vi "Write Boolean.vi"(7 "RegisterOffset":u32, 8 "error in":errorcluster, 9 "value in":bool, 10 "register name":string, 11 "session in":u32) -> (0 "error out":errorcluster, 3 "session out":u32)   [LabVIEW 2020, in "FPGA Register IO.lvlib"]
uses:
  FPGA Register IO.lvlib
  NiFpga.dll
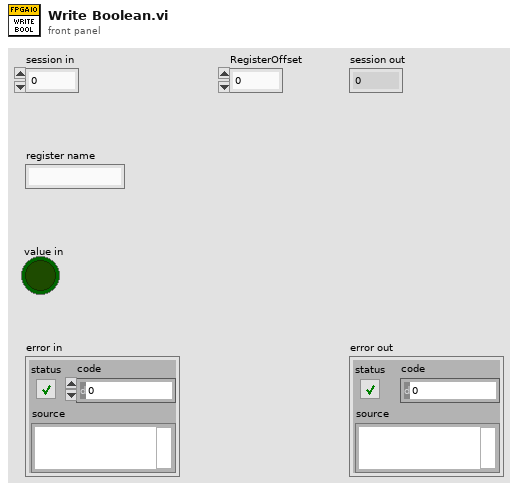
[diagram p1: front panel]
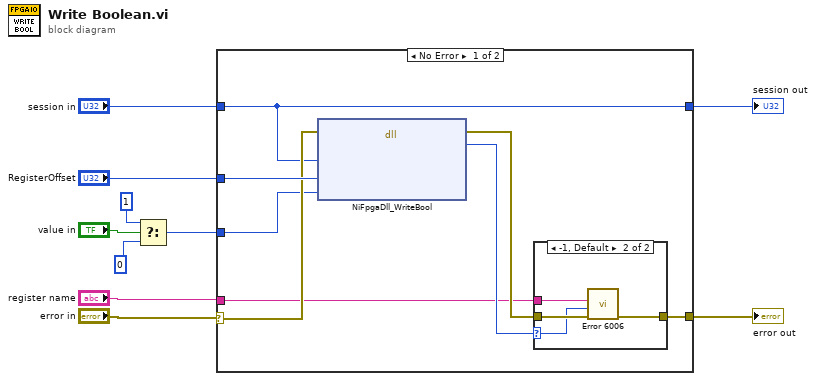
[diagram p0: block diagram]
diagram:
  n1 = Select(t=u8 1 ("value"), s="value in", f=u8 0) -> (s? t:f=w1:u8)
  n2 = case shown="No Error" "error in" {
    selector: "error in" -> [w17 w25]
    tunnel: "session in" -> [w16 w24]
    tunnel: [w11 w25] -> w10
    tunnel: "RegisterOffset" -> [w18 _]
    tunnel: [w16 w24] -> w9
    tunnel: w1 -> [w15 _]
    tunnel: "register name" -> [w12 _]
    frame No Error {
      n3 = dll-call lib="NiFpga.*" fn="NiFpgaDll_WriteBool"(error in=w17, "session"=w16, "offset"=w18, "value"=w15) -> (error out=w13:errorcluster, "status"=w14:i32)  [unwired: 5 in, 1 out]
      n4 = case shown="-1, Default" w14 {
        selector: w14 -> [_ w20]
        tunnel: w13 -> [w19 w21]
        tunnel: [w19 w23] -> w11
        tunnel: w12 -> [_ w22]
        frame 0 {
        }
        frame -1, Default {
          n5 = call "Error 6006.vi"("error in (no error)"=w21, "rio status code"=w20, "register name"=w22) -> ("error out"=w23:errorcluster)  [unwired: 8 in]
        }
      }
    }
    frame Error {
    }
  }
  "error out" <- w10
  "session out" <- w9
